vi "LV to ITX XY2 AutoPlot.vi"(8 "error in":errorcluster, 9 "Notes":string, 10 "Data (Dictionary)":T1[](array[typedef]), 11 "path":path=path "C:/") -> (0 "error out":errorcluster, 3 "file out":path)   [LabVIEW 2019, in "LV-Data.ITX.lvclass"]
doc: "Write data to ITX file. This AutoPlot VI adds commands to automatically create a graph in Igor to quickly view your data.\n\n-- path: base path to save data\n-- filename: base filename\n-- Notes: add any notes here to help you remember what experiment you did\n-- Data: Cluster array\n It is recommended that you make the first cluster an array of timestamps\n-- wavenames: Give each data array a unique name such as \"time, bias, current,...\"zz\n-- X,Y Labels: For plotting in Igor. Can be ignored.\n-- X,Y Log: Do you wan to show X or Y on Log scale in Igor?"
uses:
  LV-Data.ITX.lvclass
  ITX Commands/ITX Commands.lvclass
  LV-Data/LV-Data.lvclass
  LV-Data/Typedefs/Operation--enum.ctl
  LV-Data/Typedefs/File Type--enum.ctl
  ab6e2ebb-f122-4517-8868-94f3faca7e22.vi
  LV-Data/Typedefs/Dictionary--cluster.ctl
panel:
  in  "X,Y Log":i32[](array[numeric])
  in  "X,Y Labels":string[](array[string])=["x label", "y label"]
  # "Below are relevant for creating graphs in Igor"
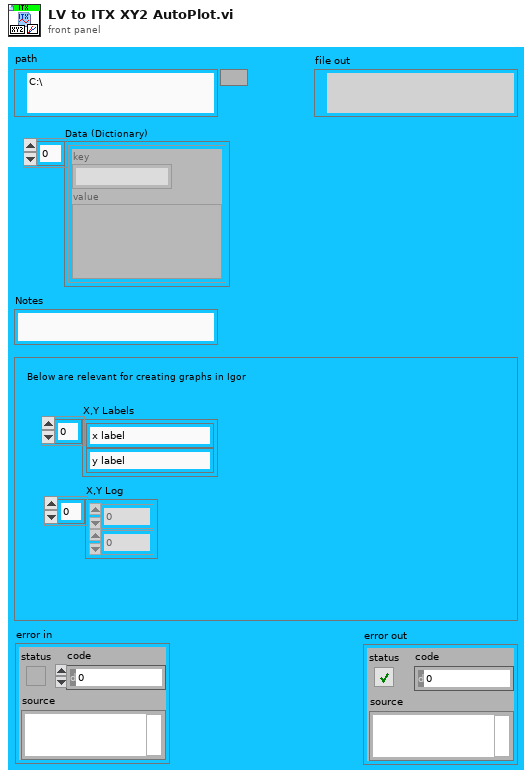
[diagram p1: front panel]
types:
  T1 = typedef "LV-Data.lvclass/Dictionary--cluster.ctl" = cluster{"key":string, "value":variant}
  T2 = typedef "LV-Data.lvclass/File Type--enum.ctl" = enum16{"DAT", "ITX", "TDMS", "VI"}
  T3 = typedef "LV-Data.lvclass/Operation--enum.ctl" = enum16{"Read", "Write", "Write + Append"}
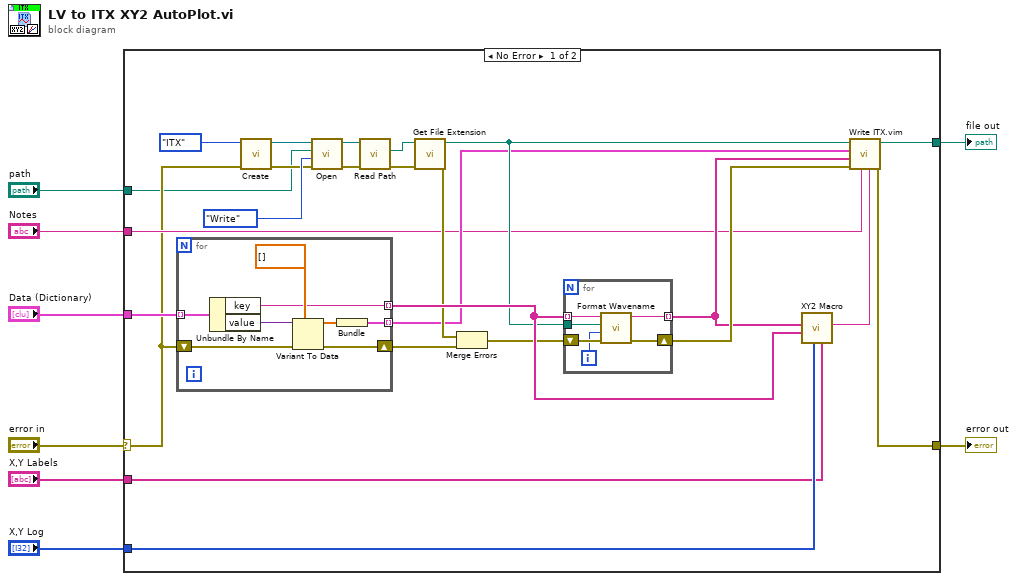
[diagram p0: block diagram]
diagram:
  n1 = case shown="No Error" "error in" {
    selector: "error in" -> [w13 w49]
    tunnel: "path" -> [w11 w48]
    tunnel: "X,Y Labels" -> [w9 _]
    tunnel: [w33 w48] -> w6
    tunnel: "X,Y Log" -> [w32 _]
    tunnel: [w27 w49] -> w4
    tunnel: "Data (Dictionary)" -> [w31 _]
    tunnel: "Notes" -> [w18 _]
    frame No Error {
      n2 = for {
        tunnel: w31 -> [w41] mode=indexing
        tunnel: [w35] -> w20 mode=indexing
        shift-right: [w36] -> w24
        shift-left: w13 -> [w39]
        tunnel: [w34] -> w30 mode=indexing
        n3 = Unbundle By Name(w41) -> ("key"=w34:string, "value"=w40:variant)
        n4 = Variant To Data(error in=w39, type=dbl[] [], Variant=w40) -> (data=w37:dbl[], error out=w36:errorcluster)
        n5 = Bundle(w37) -> (w35:cluster{dbl[]})  [unwired: 1 in]
      }
      n6 = call "Create.vi"("error in (no error)"=w13, "File Type"=File_Type--enum."ITX") -> ("error out"=w12:errorcluster, "Data out"=w14:refnum<class "LV-Data.lvclass">)  [unwired: 8 in]
      n7 = call-dynamic "Open.vi"("error in (no error)"=w12, "Operation"=Operation--enum."Write", "Path"=w11, "Data in"=w14) -> ("error out"=w17:errorcluster, "Data out"=w16:refnum<class "LV-Data.lvclass">)  [unwired: 6 in]
      n8 = call "Read Path.vi"("error in (no error)"=w17, "Data Save"=w16) -> ("error out"=w25:errorcluster, "Path"=w26:path)  [unwired: 7 in, 1 out]
      n9 = call <vilib>:"Get File Extension.vi"("error in (no error)"=w25, "file"=w26) -> ("error out"=w23:errorcluster, "dup file"=w21:path)  [unwired: 5 in, 3 out]
      n10 = Merge Errors(w23, w24) -> (w22:errorcluster)
      n11 = for {
        tunnel: w30 -> [w47] mode=indexing
        shift-right: [w45] -> w28
        shift-left: w22 -> [w46]
        tunnel: [w44] -> w19 mode=indexing
        tunnel: w21 -> [w42]
        i -> [w43]
        n12 = call "Format Wavename.vi"("error in (no error)"=w46, "Index"=w43, "Path"=w42, "Name"=w47) -> ("error out"=w45:errorcluster, "Formatted wavename"=w44:string)  [unwired: 6 in]
      }
      n13 = call "XY2 Macro.vi"("X,Y Labels"=w9, "X,Y Log"=w32, "Plot labels"=w30, "wavenames"=w19) -> ("result string"=w29:string)  [unwired: 5 in, 2 out]
      n14 = call "Write ITX.vim"("commands"=w29, "notes"=w18, "error in"=w28, "wavename"=w19, "values"=w20, "filename"=w21) -> ("error out"=w27:errorcluster, "filename out"=w33:path)  [unwired: 3 in, 1 out]
    }
    frame Error {
    }
  }
  "file out" <- w6
  "error out" <- w4
